vi "Own20261012_GetNamedUnbundlerElements.vi"() -> ()   [LabVIEW 2024]
panel:
  out "full_element_names":cluster{string[]}[](array[cluster])
  out "available_elements":string[](array[string])
  out "element_names":string[](array[string])
  out "error out":errorcluster caption="错误输出"
  in  "unbundler_id":u32
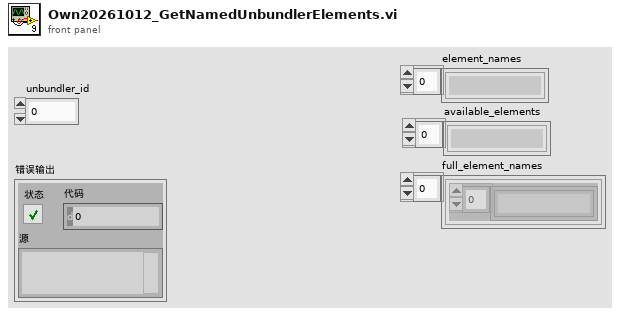
[diagram p1: front panel]
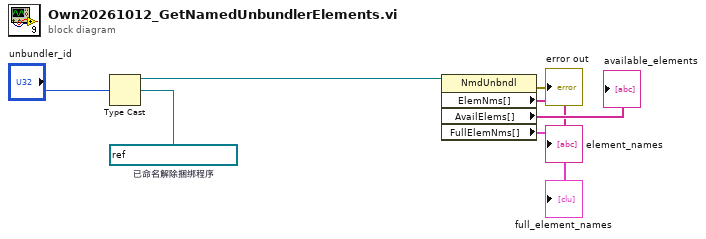
[diagram p0: block diagram]
diagram:
  w6 = refnum<vi> refnum  # 已命名解除捆绑程序
  n1 = Type Cast ("强制类型转换")(type=w6, x="unbundler_id") -> (*(type *) &x=w5:refnum<vi>)
  n2 = property on="属性节点" class="NmdUnbndl"(reference=w5) -> (error out=→"error out":errorcluster, "ElemNms[]"=→"element_names":string[], "AvailElems[]"=→"available_elements":string[], "FullElemNms[]"=→"full_element_names":cluster{string[]}[])  [unwired: 1 in, 1 out]
